vi "LabVIEW.Main.API_Test_TCP_Server.vi"() -> ()   [LabVIEW 2026]
uses:
  LabVIEW.Main.API_Test_TCP_Server_Loging_Command.ctl
  <extravilib>/ChannelInstances/Event Messenger-i32/Event Data.ctl
  <extravilib>/ChannelInstances/Event Messenger-str/Event Data.ctl
  <extravilib>/ChannelInstances/Event Messenger-bool/Event Data.ctl
  <extravilib>/ChannelInstances/Event Messenger-bool/Instantiate.vi
  <extravilib>/ChannelInstances/Event Messenger-bool/))Channel.vi
  <extravilib>/ChannelInstances/Event Messenger-i32/Instantiate.vi
  <extravilib>/ChannelInstances/Event Messenger-i32/))Channel.vi
  <extravilib>/ChannelInstances/Event Messenger-str/Instantiate.vi
  <extravilib>/ChannelInstances/Event Messenger-str/))Channel.vi
  <extravilib>/ChannelInstances/Event Messenger-str.lvlib
  <extravilib>/ChannelInstances/Event Messenger-i32.lvlib
  <extravilib>/ChannelInstances/Event Messenger-bool.lvlib
panel:
  out "Kein Fehler":errorcluster
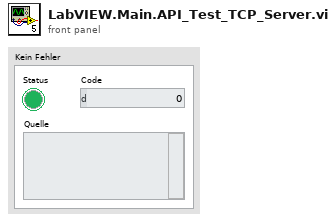
[diagram p1: front panel]
types:
  T1 = enum32{"invalid app kind", "Development System", "Run Time System", "Student Edition", "Embedded LabVIEW", "Evaluation", "Custom"}
  T2 = cluster{"Fehlercode":refnum<event-registration>, "Befehl":refnum<event-registration>, "STOP":refnum<event-registration>}
  T3 = typedef "LabVIEW.Main.API_Test_TCP_Server_Loging_Command.ctl" = enum16{"Initialize Components", "Loging", "Handel error when logging in"}
  T4 = enum32{"Invalid", "Standard", "Closed", "Hidden", "Minimized", "Maximized"}
  T5 = typedef "Event Messenger-str.lvlib/))Channel.ctl" = refnum<queue>
  T6 = cluster{"FileVersion":string, "FileMajorPart":i32, "FileMinorPart":i32, "FileBuildPart":i32, "FilePrivatePart":i32, "Language":string, "LegalCopyright":string, "FileDescription":string, "CompanyName":string, "ProductName":string, "InternalName":string}
  T7 = typedef "Event Messenger-bool.lvlib/))Channel.ctl" = refnum<queue>
  T8 = typedef "Event Messenger-i32.lvlib/))Channel.ctl" = refnum<queue>
  T9 = enum16{"Initialize Components", "Loging", "Delete Loging"}
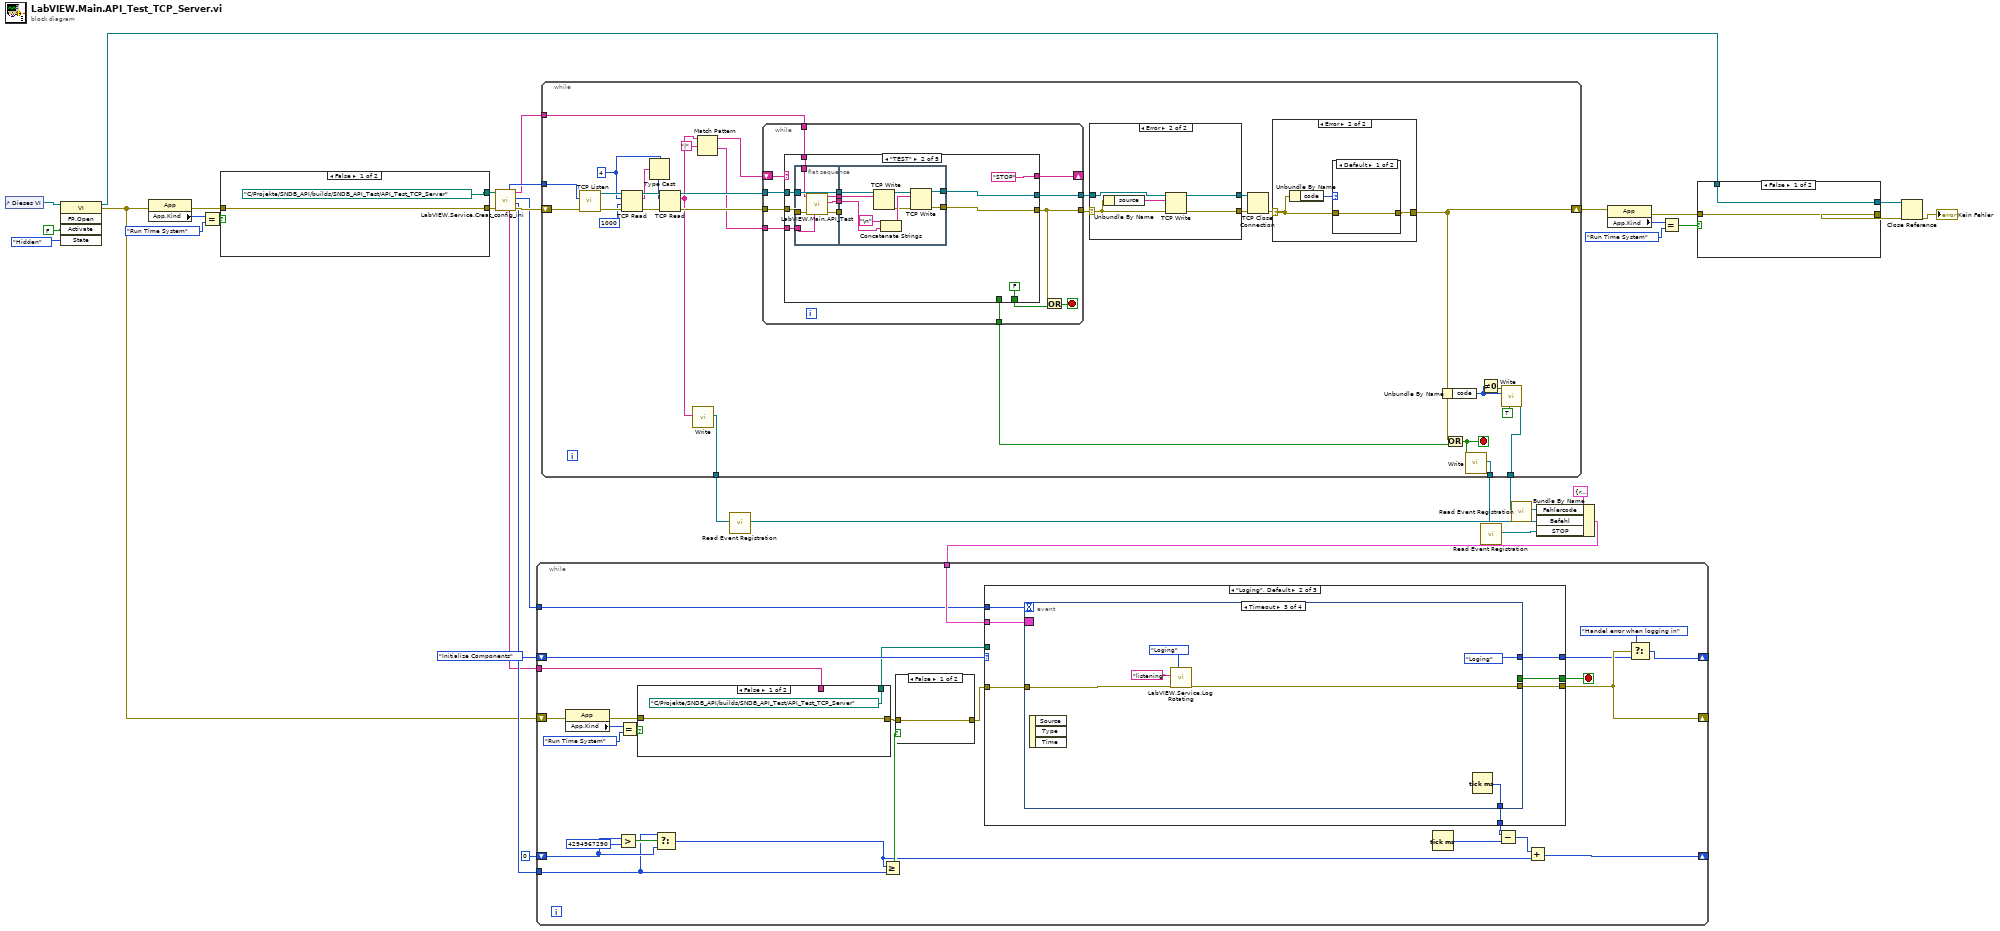
[diagram p0: block diagram]
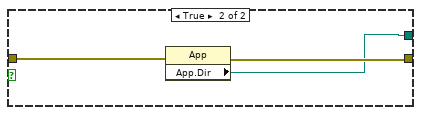
[diagram p2: hidden frame]
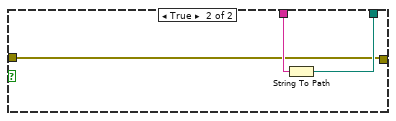
[diagram p3: hidden frame]
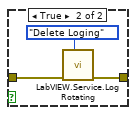
[diagram p4: hidden frame]
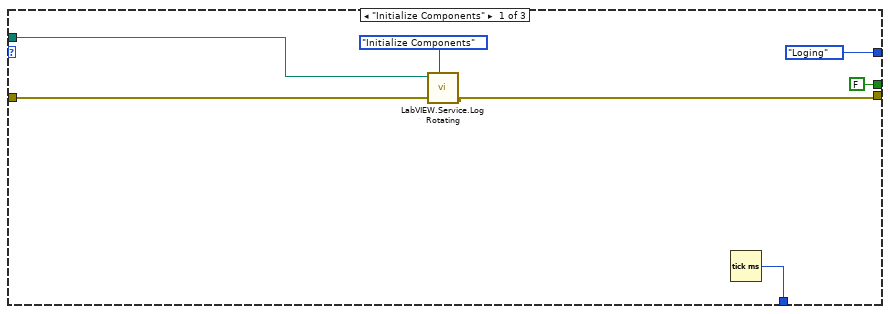
[diagram p5: hidden frame]
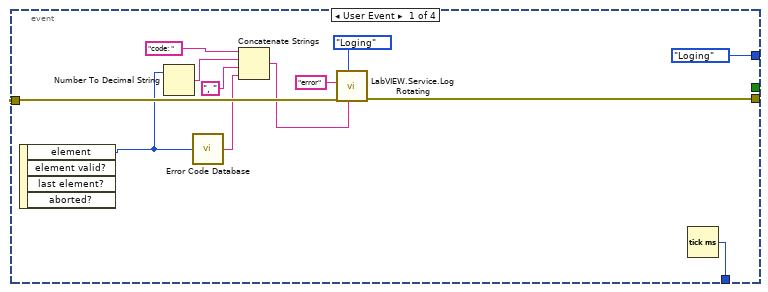
[diagram p6: hidden frame]
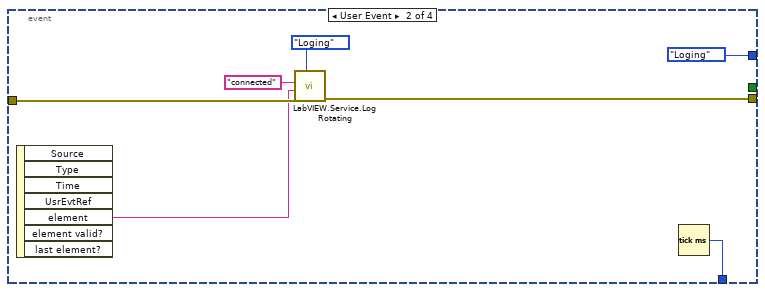
[diagram p7: hidden frame]
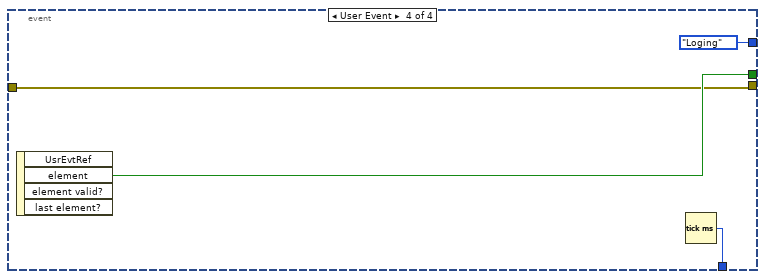
[diagram p8: hidden frame]
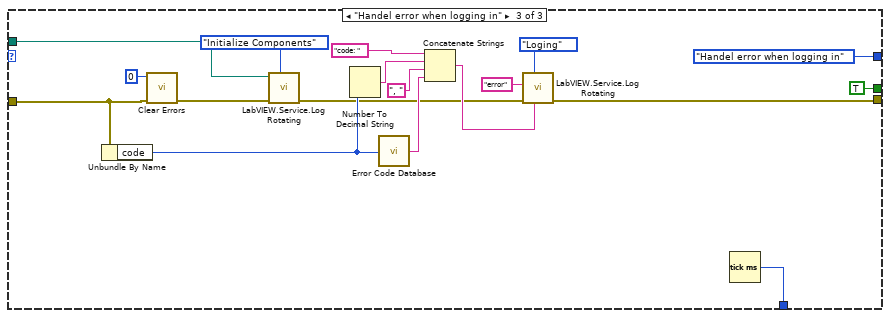
[diagram p9: hidden frame]
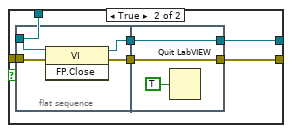
[diagram p10: hidden frame]
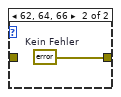
[diagram p13: hidden frame]
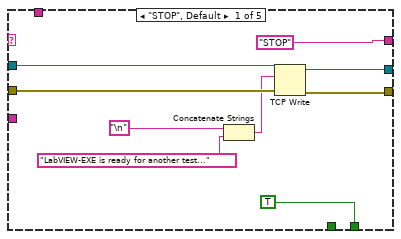
[diagram p14: hidden frame]
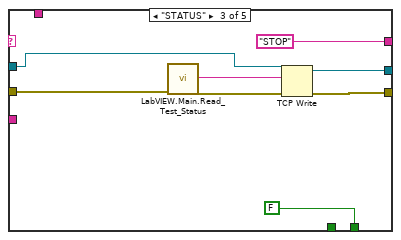
[diagram p15: hidden frame]
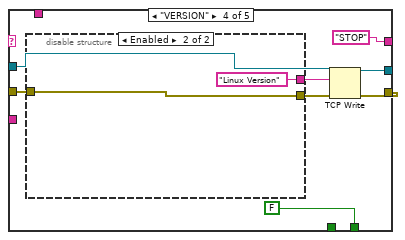
[diagram p16: hidden frame]
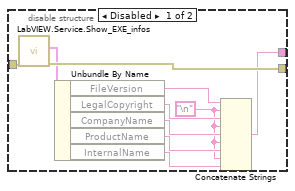
[diagram p17: hidden frame]
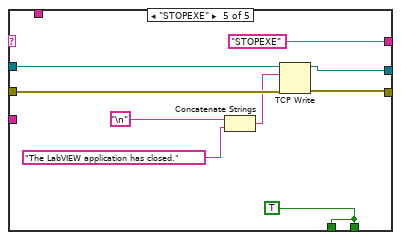
[diagram p18: hidden frame]
diagram:
  n1 = control-ref of="Dieses VI"() -> (w35:refnum<vi>)
  n2 = invoke class="VI" method="FP.Open"(reference=w35, "Activate"=FALSE ("Aktivieren?"), "State"=T4."Hidden" ("Zustand")) -> (reference out=w25:refnum<vi>, error out=w5:errorcluster)  [unwired: 2 in, 3 out]
  n3 = property class="App"(error in=w5) -> (error out=w3:errorcluster, "App.Kind"=w7:T1)  [unwired: 1 in, 1 out]
  n4 = Equal?(x=w7, y=T1."Run Time System" ("Anwendung:Typ")) -> (x = y?=w4:bool)
  n5 = case shown="False" w4 {
    tunnel: w3 -> [w36 w40]
    tunnel: [path "C:/Projekte/SNDB_API/builds/SNDB_API_Test/API_Test_TCP_Server" ("App.Dir") w38] -> w2
    tunnel: [w36 w39] -> w1
    frame False {
    }
    frame True {
      n6 = property class="App"(error in=w40) -> (error out=w39:errorcluster, "App.Dir"=w38:path)  [unwired: 1 in, 1 out]
    }
  }
  n7 = call "LabVIEW.Service.Creat_config_ini.vi"("error in (no error)"=w1, "Pfad"=w2) -> ("error out"=w13:errorcluster, "time_of_log_rotating[ms]"=w10:u32, "period_of_log_rotating[ms]"=w9:i32, "result_folder_path"=w11:string, "log_folder_path"=w8:string, "Port"=w12:u32)  [unwired: 4 in]
  n8 = while {
    shift-right: [w44] -> w32
    shift-left: w13 -> [w53]
    tunnel: [w51] -> w22
    tunnel: [w49] -> w19
    tunnel: [w48] -> w16
    tunnel: w12 -> [w42]
    tunnel: w11 -> [w41]
    stop <- w50 stop-if-true
    w65 = 4 ("Zu lesende Bytes")
    n9 = call <vilib>:"TCP Listen.vi"("error in (no error)"=w53, "port"=w42) -> ("error out"=w71:errorcluster, "connection ID"=w70:refnum<k5>)  [unwired: 5 in, 3 out]
    n10 = TCP Read(connection ID=w70, bytes to read=w65, error in (no error)=w71, 9:1000 ("Timeout in ms (25000)")) -> (connection ID out=w66:refnum<k5>, data out=w64:string, error out=w67:errorcluster)  [unwired: 1 in]
    n11 = Type Cast(type=w65, x=w64) -> (*(type *) &x=w63:i32)
    n12 = TCP Read(connection ID=w66, bytes to read=w63, error in (no error)=w67) -> (connection ID out=w58:refnum<k5>, data out=w56:string, error out=w57:errorcluster)  [unwired: 2 in]
    n13 = call <extravilib>:"Write.vi"("element"=w56) -> ("channel"=w51:T5)  [unwired: 9 in, 1 out]
    n14 = Match Pattern(string=w56, regular expression="|" ("Regulärer Ausdruck")) -> (before substring=w54:string, after substring=w43:string)  [unwired: 1 in, 2 out]
    n15 = while {
      shift-right: [w94] -> _
      shift-left: w54 -> [w95]
      tunnel: w57 -> [w93]
      tunnel: [w91] -> w62
      tunnel: [w92] -> w61
      tunnel: w58 -> [w89]
      tunnel: [w87] -> w52
      tunnel: w43 -> [w86]
      tunnel: w41 -> [w85]
      stop <- w90 stop-if-true
      n16 = case shown="\"TEST\"" w95 {
        tunnel: ["STOP" "STOP" "STOP" "STOP" "STOPEXE" ("Daten (Eingang)")] -> w94
        tunnel: w93 -> [w102 w114 w136 w144 w168]
        tunnel: [TRUE FALSE FALSE FALSE w164] -> w88
        tunnel: [w101 w108 w138 w147 w166] -> w91
        tunnel: [w100 w107 w137 w146 w167] -> w92
        tunnel: w89 -> [w99 w113 w134 w145 w169]
        tunnel: [_ _ _ _ w164] -> w87
        tunnel: w86 -> [_ w106 _ _ _]
        tunnel: w85 -> [_ w105 _ _ _]
        frame "STOP", Default {
          n17 = Concatenate Strings("\n", "LabVIEW-EXE is ready for another test..." ("Daten (Eingang)")) -> (w97:string)
          n18 = TCP Write(connection ID=w99, data in=w97, error in (no error)=w102) -> (connection ID out=w100:refnum<k5>, error out=w101:errorcluster)  [unwired: 2 out]
        }
        frame "TEST" {
          n19 = flat-sequence {
            tunnel: w114 -> [w123]
            tunnel: w113 -> [w119]
            tunnel: [w122] -> w112
            tunnel: [w121] -> w111
            tunnel: [w120] -> w110
            tunnel: [w119] -> w109
            tunnel: w106 -> [w118]
            tunnel: w105 -> [w117]
            tunnel: w112 -> [_]
            tunnel: w111 -> [w127]
            tunnel: w110 -> [w128]
            tunnel: w109 -> [w126]
            tunnel: [w125] -> w108
            tunnel: [w124] -> w107
            frame #0 {
              n20 = call "LabVIEW.Main.API_Test.vi"("Chose Server"=w118, "error in (no error)"=w123, "result_folder_path"=w117) -> ("error out"=w122:errorcluster, "Message_local_save"=w120:string, "Message_report"=w121:string)  [unwired: 6 in]
            }
            frame #1 {
              n21 = TCP Write(connection ID=w126, data in=w127) -> (connection ID out=w131:refnum<k5>, error out=w130:errorcluster)  [unwired: 1 in, 2 out]
              n22 = Concatenate Strings("\n", w128) -> (w132:string)
              n23 = TCP Write(connection ID=w131, data in=w132, error in (no error)=w130) -> (connection ID out=w124:refnum<k5>, error out=w125:errorcluster)  [unwired: 2 out]
            }
          }
        }
        frame "STATUS" {
          n24 = call "LabVIEW.Main.Read_Test_Status.vi"("error in (no error)"=w136) -> ("error out"=w135:errorcluster, "Message_report"=w133:string)  [unwired: 9 in]
          n25 = TCP Write(connection ID=w134, data in=w133, error in (no error)=w135) -> (connection ID out=w137:refnum<k5>, error out=w138:errorcluster)  [unwired: 2 out]
        }
        frame "VERSION" {
          n26 = disable-structure shown="Enabled" {
            disable-tunnel: w144 -> [w158 w160]
            disable-tunnel: [w157 w160] -> w143
            disable-tunnel: [w149 "Linux Version"] -> w142
            frame Disabled {
              w151 = "\n"
              n27 = call "LabVIEW.Service.Show_EXE_infos.vi"("error in (no error)"=w158) -> ("error out"=w157:errorcluster, "File Info Out"=w156:T6)  [unwired: 8 in, 1 out]
              n28 = Unbundle By Name(w156) -> ("FileVersion"=w155:string, "LegalCopyright"=w154:string, "CompanyName"=w153:string, "ProductName"=w152:string, "InternalName"=w150:string)
              n29 = Concatenate Strings(w155, w151, w154, w151, w153, w151, w152, w151, w150) -> (w149:string)
            }
            frame Enabled {
            }
          }
          n30 = TCP Write(connection ID=w145, data in=w142, error in (no error)=w143) -> (connection ID out=w146:refnum<k5>, error out=w147:errorcluster)  [unwired: 2 out]
        }
        frame "STOPEXE" {
          w164 = TRUE
          n31 = Concatenate Strings("\n", "The LabVIEW application has closed." ("Daten (Eingang)")) -> (w161:string)
          n32 = TCP Write(connection ID=w169, data in=w161, error in (no error)=w168) -> (connection ID out=w167:refnum<k5>, error out=w166:errorcluster)  [unwired: 2 out]
        }
      }
      n33 = Or(x=w91, y=w88) -> (x .or. y?=w90:bool)
    }
    n34 = case shown="Error" w62 {
      selector: w62 -> [w73 w74]
      tunnel: [w73 w75] -> w60
      tunnel: w61 -> [w72 w77]
      tunnel: [w72 w76] -> w59
      frame No Error {
      }
      frame Error {
        n35 = Unbundle By Name(w74) -> ("source"=w78:string)
        n36 = TCP Write(connection ID=w77, data in=w78, error in (no error)=w74) -> (connection ID out=w76:refnum<k5>, error out=w75:errorcluster)  [unwired: 2 out]
      }
    }
    n37 = TCP Close Connection(connection ID=w59, error in (no error)=w60) -> (error out=w68:errorcluster)  [unwired: 2 out]
    n38 = case shown="Error" w68 {
      selector: w68 -> [w79 w81]
      tunnel: [w79 w80] -> w44
      frame No Error {
      }
      frame Error {
        n39 = Unbundle By Name(w81) -> ("code"=w82:i32)
        n40 = case shown="Default" w82 {
          tunnel: w81 -> [w83 _]
          tunnel: [w83 w84] -> w80
          frame Default {
          }
          frame 62, 64, 66 {
            w84 = errorcluster {"status"=FALSE, "code"=0, "source"=""}  # Kein Fehler
          }
        }
      }
    }
    n41 = Unbundle By Name(w44) -> ("code"=w47:i32)
    n42 = Or(x=w44, y=w52) -> (x .or. y?=w50:bool)
    n43 = call <extravilib>:"Write.vi"("element"=w50) -> ("channel"=w48:T7)  [unwired: 9 in, 1 out]
    n44 = Not Equal To 0?(x=w47) -> (x != 0?=w46:bool)
    n45 = call <extravilib>:"Write.vi"("high priority? (F)"=TRUE, "element"=w47, "element valid? (T)"=w46) -> ("channel"=w49:T8)  [unwired: 7 in, 1 out]
  }
  n46 = call <extravilib>:"Read Event Registration.vi"("channel"=w22) -> ("event registration refnum"=w20:refnum<event-registration>)  [unwired: 10 in]
  n47 = call <extravilib>:"Read Event Registration.vi"("channel"=w16) -> ("event registration refnum"=w15:refnum<event-registration>)  [unwired: 10 in]
  n48 = call <extravilib>:"Read Event Registration.vi"("channel"=w19) -> ("event registration refnum"=w18:refnum<event-registration>)  [unwired: 10 in]
  n49 = Bundle By Name(cluster=T2 {"Fehlercode"=refnum, "Befehl"=refnum, "STOP"=refnum}, "Fehlercode"=w18, "Befehl"=w20, "STOP"=w15) -> (w17:T2)
  n50 = while {
    shift-right: [w186] -> _
    shift-left: LabVIEW.Main.API_Test_TCP_Server_Loging_Command."Initialize Components" ("Command") -> [w196]
    tunnel: w17 -> [w195]
    shift-right: [w191] -> _
    shift-left: u32 0 -> [w172]
    shift-right: [w188] -> _
    shift-left: w5 -> [w179]
    tunnel: w10 -> [w170]
    tunnel: w9 -> [w176]
    tunnel: w8 -> [w175]
    stop <- w189 stop-if-true
    n51 = property class="App"(error in=w179) -> (error out=w178:errorcluster, "App.Kind"=w181:T1)  [unwired: 1 in, 1 out]
    n52 = Greater?(x=w172, y=u32 4294967290) -> (0:w173:bool)
    n53 = Equal?(x=w181, y=T1."Run Time System" ("Anwendung:Typ")) -> (x = y?=w177:bool)
    n54 = case shown="False" w177 {
      tunnel: [w198 w199] -> w183
      tunnel: [path "C:/Projekte/SNDB_API/builds/SNDB_API_Test/API_Test_TCP_Server" ("App.Dir") w201] -> w182
      tunnel: w178 -> [w198 w199]
      tunnel: w175 -> [_ w200]
      frame False {
      }
      frame True {
        n55 = String To Path(string=w200) -> (path=w201:path)
      }
    }
    n56 = Select(t=w170, s=w173, f=w172) -> (s? t:f=w171:u32)
    n57 = Greater Or Equal?(x=w171, y=w170) -> (x >= y?=w190:bool)
    n58 = case shown="False" w190 {
      tunnel: w183 -> [w202 w204]
      tunnel: [w202 w203] -> w184
      frame False {
      }
      frame True {
        n59 = call "LabVIEW.Service.Log Rotating.vi"("Command"=T9."Delete Loging", "error in (no error)"=w204) -> ("error out"=w203:errorcluster)  [unwired: 9 in]
      }
    }
    n60 = case shown="\"Loging\", Default" w196 {
      tunnel: w184 -> [w211 w215 w253]
      tunnel: [w210 w219 w256] -> w188
      tunnel: [LabVIEW.Main.API_Test_TCP_Server_Loging_Command."Loging" ("Command") w218 LabVIEW.Main.API_Test_TCP_Server_Loging_Command."Handel error when logging in" ("Command")] -> w187
      tunnel: w195 -> [_ w214 _]
      tunnel: [FALSE ("element") w217 TRUE ("element")] -> w189
      tunnel: [w208 w216 w255] -> w194
      tunnel: w182 -> [w206 _ w249]
      tunnel: w176 -> [_ w213 _]
      frame "Initialize Components" {
        n61 = call "LabVIEW.Service.Log Rotating.vi"("Command"=T9."Initialize Components", "error in (no error)"=w211, "Pfad"=w206) -> ("error out"=w210:errorcluster)  [unwired: 8 in]
        n62 = Tick Count (ms)() -> (millisecond timer value=w208:u32)
      }
      frame "Loging", Default {
        n63 = event shown="[2] Timeout" {
          selector: w214 -> [_ _ _ _]
          dyn-events: _ -> [_ _ _ _]
          timeout: w213 -> [_ _ _ _]
          tunnel: w215 -> [w230 w236 w244 w247]
          tunnel: [w231 w235 w243 w247] -> w219
          tunnel: [LabVIEW.Main.API_Test_TCP_Server_Loging_Command."Loging" ("Command") LabVIEW.Main.API_Test_TCP_Server_Loging_Command."Loging" ("Command") LabVIEW.Main.API_Test_TCP_Server_Loging_Command."Loging" ("Command") LabVIEW.Main.API_Test_TCP_Server_Loging_Command."Loging" ("Command")] -> w218
          tunnel: [_ _ _ w248] -> w217
          tunnel: [w228 w233 w241 w246] -> w216
          event User Event {
            n64 = event-data() -> ("element"=w225:i32)  [unwired: 1 in, 3 out]
            n65 = Number To Decimal String(number=w225) -> (decimal integer string=w223:string)  [unwired: 1 in]
            n66 = call <vilib>:"Error Code Database.vi"("Error Code"=w225) -> ("Error Text"=w221:string)
            n67 = Concatenate Strings("code: " ("String"), w223, ", " ("String"), w221) -> (w220:string)
            n68 = call "LabVIEW.Service.Log Rotating.vi"("description"=w220, "Command"=T9."Loging", "error in (no error)"=w230, "status"="error") -> ("error out"=w231:errorcluster)  [unwired: 7 in]
            n69 = Tick Count (ms)() -> (millisecond timer value=w228:u32)
          }
          event User Event {
            n70 = event-data() -> ("element"=w232:string)  [unwired: 1 in, 6 out]
            n71 = call "LabVIEW.Service.Log Rotating.vi"("Command"=T9."Loging", "error in (no error)"=w236, "command"=w232, "status"="connected") -> ("error out"=w235:errorcluster)  [unwired: 7 in]
            n72 = Tick Count (ms)() -> (millisecond timer value=w233:u32)
          }
          event Timeout {
            n73 = event-data() -> ()  [unwired: 1 in, 3 out]
            n74 = call "LabVIEW.Service.Log Rotating.vi"("Command"=T9."Loging", "error in (no error)"=w244, "status"="listening") -> ("error out"=w243:errorcluster)  [unwired: 8 in]
            n75 = Tick Count (ms)() -> (millisecond timer value=w241:u32)
          }
          event User Event {
            n76 = event-data() -> ("element"=w248:bool)  [unwired: 1 in, 3 out]
            n77 = Tick Count (ms)() -> (millisecond timer value=w246:u32)
          }
        }
      }
      frame "Handel error when logging in" {
        n78 = Unbundle By Name(w253) -> ("code"=w257:i32)
        n79 = call <vilib>:"Clear Errors.vi"("error in (no error)"=w253, "specific error code to clear (0: all)"=0) -> ("error out"=w251:errorcluster)  [unwired: 4 in, 1 out]
        n80 = call "LabVIEW.Service.Log Rotating.vi"("Command"=T9."Initialize Components", "error in (no error)"=w251, "Pfad"=w249) -> ("error out"=w250:errorcluster)  [unwired: 8 in]
        n81 = Number To Decimal String(number=w257) -> (decimal integer string=w261:string)  [unwired: 1 in]
        n82 = call <vilib>:"Error Code Database.vi"("Error Code"=w257) -> ("Error Text"=w259:string)
        n83 = Concatenate Strings("code: " ("String"), w261, ", " ("String"), w259) -> (w258:string)
        n84 = call "LabVIEW.Service.Log Rotating.vi"("description"=w258, "Command"=T9."Loging", "error in (no error)"=w250, "status"="error") -> ("error out"=w256:errorcluster)  [unwired: 7 in]
        n85 = Tick Count (ms)() -> (millisecond timer value=w255:u32)
      }
    }
    n86 = Tick Count (ms)() -> (millisecond timer value=w193:u32)
    n87 = Subtract(x=w194, y=w193) -> (x-y=w192:u32)
    n88 = Add(x=w192, y=w171) -> (x+y=w191:u32)
    n89 = Select(t=LabVIEW.Main.API_Test_TCP_Server_Loging_Command."Handel error when logging in", s=w188, f=w187) -> (s? t:f=w186:T3)
  }
  n90 = property class="App"(error in=w32) -> (error out=w28:errorcluster, "App.Kind"=w31:T1)  [unwired: 1 in, 1 out]
  n91 = Equal?(x=w31, y=T1."Run Time System" ("Anwendung:Typ")) -> (x = y?=w29:bool)
  n92 = case shown="False" w29 {
    tunnel: w28 -> [w267 w274]
    tunnel: [w267 w273] -> w27
    tunnel: [w268 w272] -> w26
    tunnel: w25 -> [w268 w271]
    frame False {
    }
    frame True {
      n93 = flat-sequence {
        tunnel: w274 -> [w278]
        tunnel: w271 -> [w275]
        tunnel: [w277] -> w270
        tunnel: [w276] -> w269
        tunnel: [w280] -> w272
        tunnel: [w281] -> w273
        tunnel: w270 -> [w281]
        tunnel: w269 -> [w280]
        frame #0 {
          n94 = invoke class="VI" method="FP.Close"(reference=w275, error in=w278) -> (reference out=w276:refnum<vi>, error out=w277:errorcluster)  [unwired: 1 in, 1 out]
        }
        frame #1 {
          n95 = Quit LabVIEW(quit? (T)=TRUE ("Beenden? (T)")) -> ()
        }
      }
    }
  }
  n96 = Close Reference(reference=w26, error in (no error)=w27) -> (error out=→"Kein Fehler":errorcluster)
